vi "Dequeue Message Data.vi"(8 "error in (no error)":errorcluster, 11 "Message Queue":refnum<queue>) -> (0 "error out":errorcluster, 1 "Data":variant, 2 "Message":string, 3 "dup Message Queue":refnum<queue>)   [LabVIEW 2021]
uses:
  Type defs/Message cluster.ctl
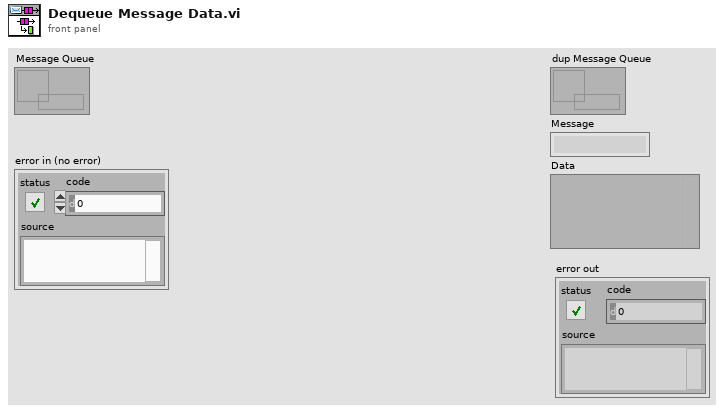
[diagram p1: front panel]
types:
  T1 = typedef "Message cluster.ctl" = cluster{"Message":string, "Data":variant}
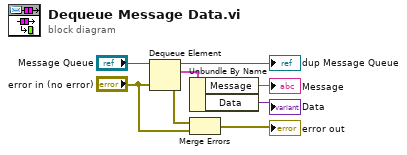
[diagram p0: block diagram]
diagram:
  n1 = Dequeue Element(queue="Message Queue", error in (no error)="error in (no error)") -> (queue out=→"dup Message Queue":refnum<queue>, element=w6:T1, error out=w3:errorcluster)  [unwired: 1 in, 1 out]
  n2 = Unbundle By Name(w6) -> ("Message"=→"Message":string, "Data"=→"Data":variant)
  n3 = Merge Errors(w3, "error in (no error)") -> (→"error out":errorcluster)
